vi "ComputeCellRect.vi"(0 "border X":i32=3, 1 "Border Y":i32=3, 2 "cell width":i32, 3 "cell height":i32, 4 "col idx":i32, 5 "line idx":i32) -> (18 "subset rect":cluster{i32, i32, i32, i32})   [LabVIEW 2026]
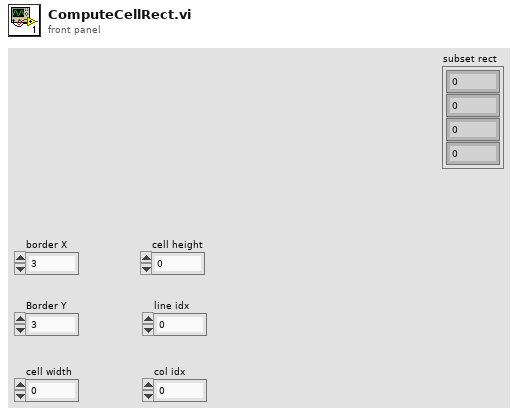
[diagram p1: front panel]
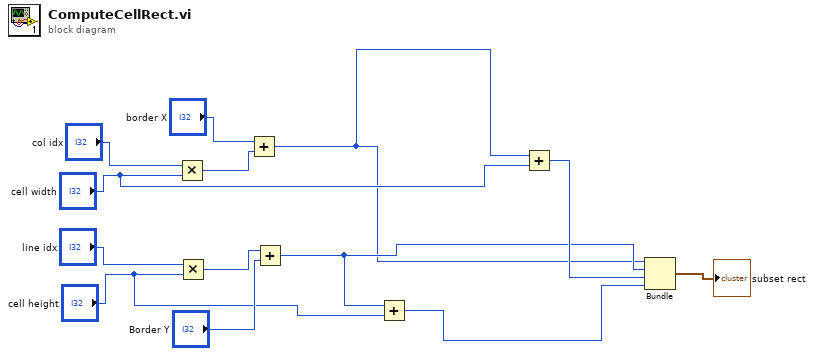
[diagram p0: block diagram]
diagram:
  n1 = Multiply(x="col idx", y="cell width") -> (x*y=w12:i32)
  n2 = Multiply(x="line idx", y="cell height") -> (x*y=w9:i32)
  n3 = Add(x="border X", y=w12) -> (x+y=w2:i32)
  n4 = Add(x=w9, y="Border Y") -> (x+y=w3:i32)
  n5 = Add(x=w3, y="cell height") -> (x+y=w5:i32)
  n6 = Add(x=w2, y="cell width") -> (x+y=w4:i32)
  n7 = Bundle(w2, w3, w4, w5) -> (→"subset rect":cluster{i32, i32, i32, i32})  [unwired: 1 in]
